vi "getStringBounds.vi"(0 "reference":refnum<class "Graphics.lvclass">, 1 "text":string, 2 "fontType":T2, 3 "font":T3, 5 "error in (no error)":errorcluster) -> (14 "reference out":refnum<class "Graphics.lvclass">, 15 "bounds":T1 {"height" format="%.2f"; "width" format="%.2f"; "y" format="%.2f"; "x" format="%.2f"}, 19 "error out":errorcluster)   [LabVIEW 2020, in "Graphics.lvclass"]
doc: "Gets the size of a string"
uses:
  <resource>/Framework/Providers/Open_GDS/UML/Graphics_class/Graphics.lvclass
  <resource>/Framework/Providers/Open_GDS/UML/Graphics_class/FontType.ctl
  <resource>/Framework/Providers/Open_GDS/UML/Graphics_class/LvFontType.ctl
  <resource>/Framework/Providers/Open_GDS/UML/General/Rectangle/Rectangle Rectangle2D.ctl
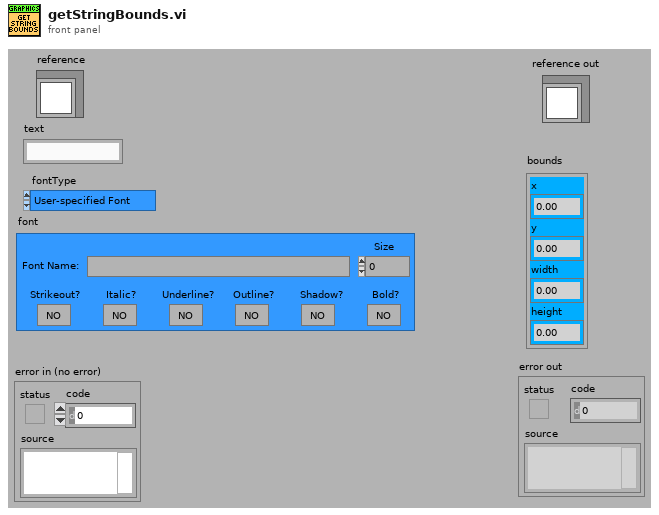
[diagram p1: front panel]
types:
  T1 = typedef "Rectangle Rectangle2D.ctl" = cluster{"x":dbl, "y":dbl, "width":dbl, "height":dbl}
  T2 = typedef "Graphics.lvclass/LvFontType.ctl" = enum16{"User-specified Font", "Application Font", "System Font", "Dialog Font"}
  T3 = typedef "Graphics.lvclass/FontType.ctl" = cluster{"Font Name:":string, "Size":i16, "Strikeout?":bool, "Italic?":bool, "Underline?":bool, "Outline?":bool, "Shadow?":bool, "Bold?":bool}
  T4 = typedef "Graphics.lvclass/ObjectAttributes.ctl" = cluster{"drawColor":u32, "backgroundColor":u32, "font":T3, "fontType":T2, "picture":picture, "stroke":T5, "scaleX":dbl, "scaleY":dbl, "screenRef":refnum<vi>, "offsetX":dbl, "offsetY":dbl}
  T5 = typedef "Graphics.lvclass/StrokeType.ctl" = enum16{"USE_DEFAULT", "SOLID", "DOTTED"}
  T6 = cluster{"left":i16, "top":i16, "right":i16, "bottom":i16}
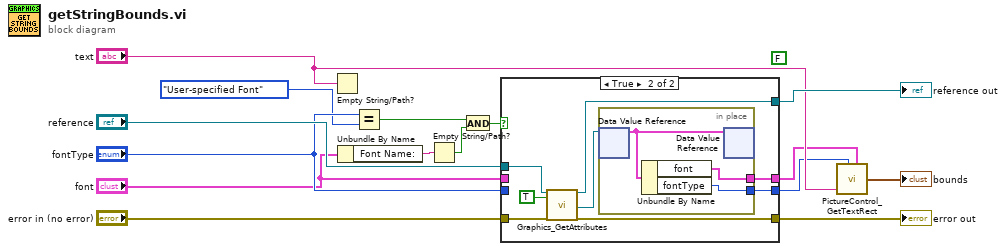
[diagram p0: block diagram]
diagram:
  (unwired) FALSE
  n1 = Empty String/Path?(string/path="text") -> ()  [unwired: 1 out]
  n2 = Unbundle By Name("font") -> ("Font Name:"=w6:string)
  n3 = Equal?(x="fontType", y=LvFontType."User-specified Font" ("fontType")) -> (x = y?=w5:bool)
  n4 = Empty String/Path?(string/path=w6) -> (empty?=w4:bool)
  n5 = And(x=w5, y=w4) -> (x .and. y?=w3:bool)
  n6 = case shown="True" w3 {
    tunnel: [w19 w22] -> w2
    tunnel: [w18 w23] -> w1
    tunnel: "font" -> [w18 _]
    tunnel: "fontType" -> [w19 _]
    tunnel: "reference" -> [w17 w27]
    tunnel: [w17 w26] -> w12
    tunnel: "error in (no error)" -> [w16 w25]
    tunnel: [w16 w24] -> w13
    frame False {
    }
    frame True {
      n7 = call <resource>:"Graphics_GetAttributes.vi"("reference in"=w27, "OnlyGetDvrReference(False)"=TRUE, "error in (no error)"=w25) -> ("reference out"=w26:refnum<class "Graphics.lvclass">, "DataRef"=w20:refnum<data-value>, "error out"=w24:errorcluster)  [unwired: 14 out]
      n8 = in-place {
        in-place-border: [w30] -> w23
        in-place-border: [w29] -> w22
        n9 = in-place-dvr #1(w20) -> (w28:T4)  [unwired: 1 out]
        n10 = Unbundle By Name(w28) -> ("font"=w30:T3, "fontType"=w29:T2)
        n11 = in-place-dvr #1(w28) -> ()  [unwired: 2 out]
      }
    }
  }
  "reference out" <- w12
  "error out" <- w13
  n12 = call <resource>:"PictureControl_GetTextRect.vi"("desired font(Application)"=w2, "text"="text", "[user-specified font]"=w1) -> ("rect"=→"bounds":T6)  [unwired: 6 in]
